vi "lvmcp_proplink.vi"() -> ()   [LabVIEW 2015]
panel:
  out "error out":errorcluster
  in  "control":refnum<vi>
  in  "reference":refnum<vi>
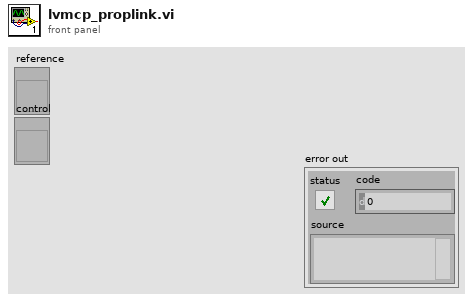
[diagram p1: front panel]
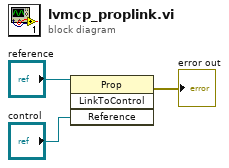
[diagram p0: block diagram]
diagram:
  n1 = invoke class="Prop" method="LinkToControl"(reference="reference", "Reference"="control") -> (error out=→"error out":errorcluster)  [unwired: 2 in, 3 out]
